vi "Run Tests - When Tests Provided - Returns Test Results For Same Test Cases.vi"(10 "Test Results":refnum<class "Test Result.lvclass">[](array[class]), 11 "Test Cases":refnum<class "LVUnit Test Case.lvclass">[](array[class])) -> (0 "error out":errorcluster)   [LabVIEW 2017, in "LVUnit Test Executor.Tests.lvlib"]
uses:
  LVUnit Test Executor.Tests.lvlib
  LVUnit Test Case/LVUnit Test Case.lvclass
  C:/Users/pasca/Projects/Home/lvunit/Test Case/Test Case.lvclass
  Test Result/Test Result.lvclass
  LVUnit Test Executor/LVUnit Test Executor.lvclass
  Test Result/Test Result.lvclass/Test Result.ctl
  Test Result/Get Test Case.vi
  Test Case/Test Case.lvclass
  <vilib>/PNR/Transparent Assertions/Transparent Assertions/Transparent Assertions.lvlib
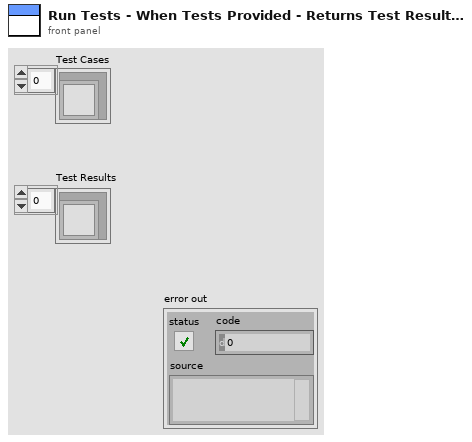
[diagram p1: front panel]
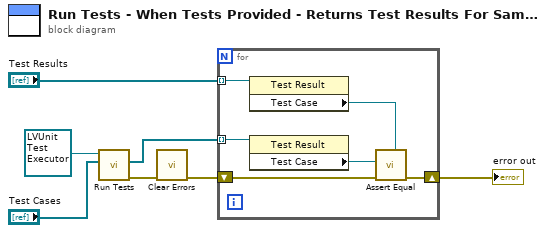
[diagram p0: block diagram]
diagram:
  n1 = call-dynamic "Run Tests.vi"("Test Cases"="Test Cases", "LVUnit Test Executor in"=refnum<class "LVUnit Test Executor.lvclass"> refnum ("LVUnit Test Executor")) -> ("error out"=w5:errorcluster, "Test Results"=w3:refnum<class "Test Result.lvclass">[])  [unwired: 7 in, 1 out]
  n2 = call <vilib>:"Clear Errors.vi"("error in (no error)"=w5) -> ("error out"=w1:errorcluster)  [unwired: 5 in, 1 out]
  n3 = for {
    tunnel: w3 -> [w9] mode=indexing
    tunnel: "Test Results" -> [w11] mode=indexing
    shift-right: [w13] -> w4
    shift-left: w1 -> [w12]
    n4 = property class="Test Result"(reference=w11) -> ("Test Case"=w10:refnum<class "Test Case.lvclass">)  [unwired: 1 in, 2 out]
    n5 = property class="Test Result"(reference=w9) -> ("Test Case"=w8:refnum<class "Test Case.lvclass">)  [unwired: 1 in, 2 out]
    n6 = call <vilib>:"Assert Equal.vi"("Expected"=w10, "error in (no error)"=w12, "Actual"=w8) -> ("error out"=w13:errorcluster)  [unwired: 8 in]
  }
  "error out" <- w4
